vi "SCADA_Master_Controller.vis.vi"() -> ()   [LabVIEW 2026]
uses:
  <vilib>/httpClient/POSTBuffer.vi
  <vilib>/httpClient/LabVIEWHTTPClient.lvlib
panel:
  in  "stop":bool
  out "value":T1
  in  "Cluster":T2
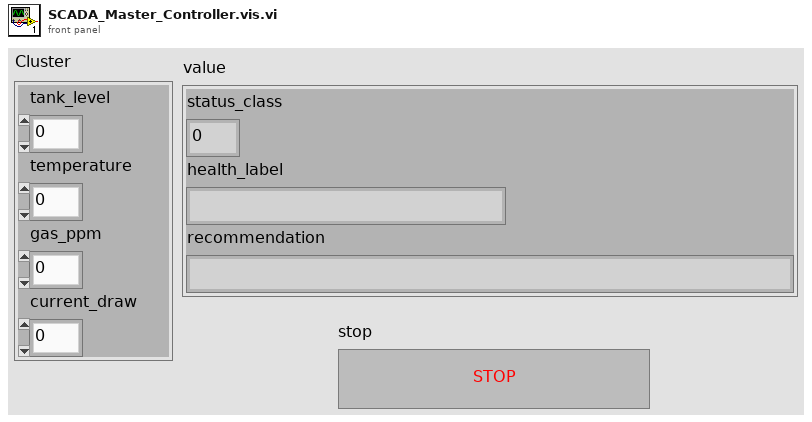
[diagram p1: front panel]
types:
  T1 = cluster{"status_class":dbl, "health_label":string, "recommendation":string}
  T2 = cluster{"tank_level":dbl, "temperature":dbl, "gas_ppm":dbl, "current_draw":dbl}
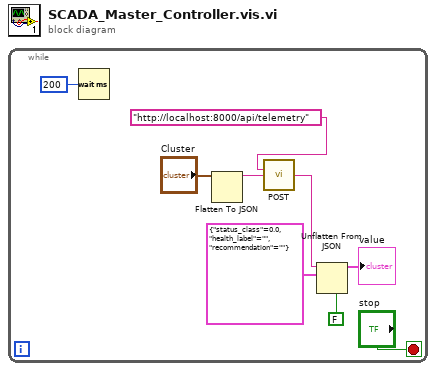
[diagram p0: block diagram]
diagram:
  n1 = while {
    stop <- "stop" stop-if-true
    n2 = Wait (ms)(milliseconds to wait=u32 200) -> ()  [unwired: 1 out]
    n3 = Flatten To JSON(anything="Cluster") -> (JSON string=w8:string)  [unwired: 2 in, 1 out]
    n4 = call-poly <vilib>:"POST.vi"("url"="http://localhost:8000/api/telemetry", "buffer"=w8) -> ("body"=w5:string)  [unwired: 10 in, 3 out]
    n5 = Unflatten From JSON(JSON string=w5, type and defaults=T1 {"status_class"=0.0, "health_label"="", "recommendation"=""}, strict validation? (F)=FALSE) -> (value=→"value":T1)  [unwired: 4 in, 1 out]
  }
